vi "Laser Power Control.vi"(7 "Calling VI Ref":refnum<vi>) -> ()   [LabVIEW 2016]
uses:
  Laser Power Control Type Defs/Laser Power Ctrl Main Control.ctl
  Laser Power Control Type Defs/Laser Power Ctrl Setup.ctl
  Hardware Configuration/Hardware Configuration Controls/Device Type.ctl
  <vilib>/Utility/miscctls.llb/LVPointTypeDef.ctl
  Laser Power Control Type Defs/Laser Power Ctrl Settings.ctl
  Hardware Configuration/Hardware Configuration Controls/Device Function.ctl
  Laser Power Control Type Defs/Laser Power Ctrl Notifier Type.ctl
  Laser Power Control Type Defs/Laser Power Ctrl Actions.ctl
  Laser Power Control Type Defs/Laser Power Ctrl Base Type.ctl
  Laser Power Control Type Defs/Laser Power Ctrl Type.ctl
  Device Library/Lasers/Laser Controls/Laser Actions.ctl
  Device Library/AOTFs/AOTF Controls/AOTF Actions.ctl
  Device Library/Lasers/External Power Control/External Power Control Type Defs/External Power Actions.ctl
  Device Manager/Common Device Queue/Common Device Controls/Common Device Actions.ctl
  <vilib>/regexp/Match Regular Expression.xnode
panel:
  in  "Manual Laser Ctrl.":bool
  out "Tab Control":enum32{"Power Adjust", "Setup"}(tab)
  in  "Power Ctrl 04":T1={"Wavelength (nm)"=0, "Active"=TRUE, "Power"=0.0, "Power Slider"=0, "Ctrl Status"=""} {"Power Slider" scale=0.0..100.0}
  in  "Power Ctrl 03":T1={"Wavelength (nm)"=0, "Active"=TRUE, "Power"=0.0, "Power Slider"=0, "Ctrl Status"=""} {"Power Slider" scale=0.0..100.0}
  in  "Power Ctrl 02":T1={"Wavelength (nm)"=0, "Active"=TRUE, "Power"=0.0, "Power Slider"=0, "Ctrl Status"=""} {"Power Slider" scale=0.0..100.0}
  in  "Power Ctrl 01":T1={"Wavelength (nm)"=0, "Active"=TRUE, "Power"=0.0, "Power Slider"=0, "Ctrl Status"=""} {"Power Slider" scale=0.0..100.0}
  in  "Power Ctrl 00":T1={"Wavelength (nm)"=0, "Active"=TRUE, "Power"=0.0, "Power Slider"=0, "Ctrl Status"=""} {"Power Slider" scale=0.0..100.0}
  in  "Power Setup 04":T2 {"Power Control Mode" items=["Direct", "AOTF", "External Ctrl"]}
  in  "Power Setup 03":T2 {"Power Control Mode" items=["Direct", "AOTF", "External Ctrl"]}
  in  "Power Setup 02":T2 {"Power Control Mode" items=["Direct", "AOTF", "External Ctrl"]}
  in  "Power Setup 01":T2 {"Power Control Mode" items=["Direct", "AOTF", "External Ctrl"]}
  in  "Power Setup 00":T2 {"Power Control Mode" items=["Direct", "AOTF", "External Ctrl"]}
  in  "Power Ctrl Setup":bool=TRUE
  in  "Quit":bool
  # "Ctrl Status:"
  # "Ctrl Status:"
  # "Ctrl Status:"
  # "Ctrl Status:"
  # "Ctrl Status:"
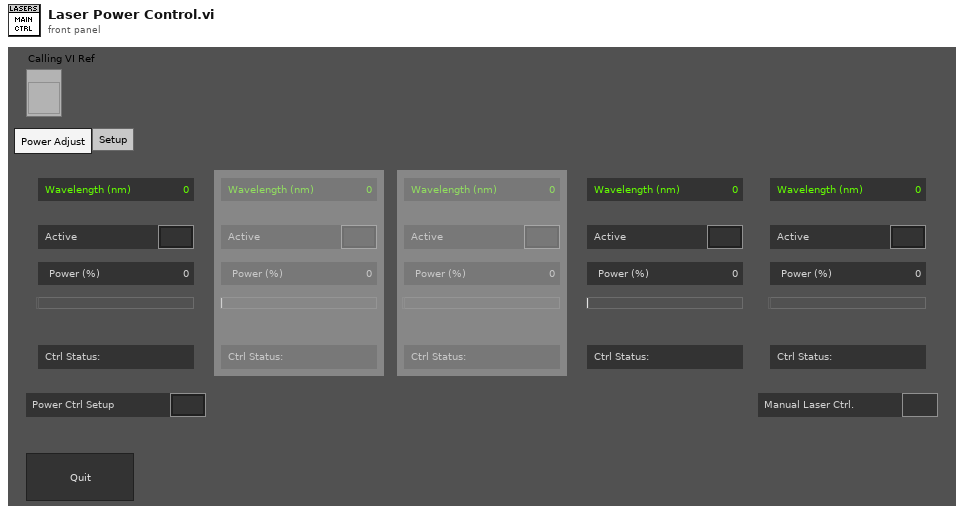
[diagram p1: front panel]
types:
  T1 = typedef "Laser Power Ctrl Main Control.ctl" = cluster{"Wavelength (nm)":u16, "Active":bool, "Power":dbl, "Power Slider":u8, "Ctrl Status":string}
  T2 = typedef "Laser Power Ctrl Setup.ctl" = cluster{"Wavelength (nm)":u16, "Power Control Mode":u16, "Ext Settings":bool, "Ext. Ctrl":string, "Pop Out":bool}
  T3 = typedef "Device Function.ctl" = enum16{"Primary", "Secondary", "Overview", "Wide Field Drift Correction", "642 nm Excitation", "560 nm Excitation", "940 nm Excitation", "546 nm Excitation", "488 nm Excitation", "405 nm Excitation", "Objective Drift Correction", "4Pi Objective Lock", "Objective XY", "Objective Z", "Sample XY", "Sample Coarse Z", "Sample Z", "4Pi Lower", "4Pi Upper", "Mojo", "Adj Cavity", "Line Scanning", "Alert"}
  T4 = typedef "Device Type.ctl" = enum16{"AOTF", "Camera", "Deformable Mirror", "Laser", "Shutter", "Stage", "Waveform", "FPGA", "Email", "Filter Wheel"}
  T5 = typedef "Laser Power Ctrl Settings.ctl" = cluster{"Wavelength":u16, "Ctrl Mode":u16, "Ext Ctrl Path":string, "Settings":string[]}
  T6 = enum16{"Always On", "Always Off", "Off While Running"}
  T7 = typedef "LVPointTypeDef.ctl" = cluster{"Horizontal":i16, "Vertical":i16}
  T8 = typedef "LVRectTypeDef.ctl" = cluster{"Left":i16, "Top":i16, "Right":i16, "Bottom":i16}
  T9 = typedef "LVBoundsTypeDef.ctl" = cluster{"Width":u32, "Height":u32}
  T10 = typedef "Laser Power Ctrl Base Type.ctl" = cluster{"Active":bool, "Power":dbl, "Ctrl Mode":u16}
  T11 = typedef "Laser Power Ctrl Actions.ctl" = enum16{"Exit Loop", "Active", "Power Adj", "All Active On", "All Active Off", "Quit"}
  T12 = typedef "Laser Power Ctrl Notifier Type.ctl" = cluster{"Actions":T11, "Wavelength":u16, "Wavelengths":u16[], "Power Ctrl":T10[]}
  T13 = typedef "Laser Actions.ctl" = enum16{"Error Check", "Set On/Off", "Set Power", "Set Parameter", "Get Power", "Get Status", "Get Parameter", "Quit"}
  T14 = typedef "AOTF Actions.ctl" = enum16{"Error Check", "Blank", "Line On/Off", "Set Power", "Status", "Quit"}
  T15 = typedef "External Power Actions.ctl" = enum16{"Line On/Off", "Set Power", "Set Ctrl Parameters", "Quit"}
  T16 = enum8{"Enabled", "Disabled", "Disabled and Grayed Out"}
  T17 = typedef "Laser Power Ctrl Type.ctl" = enum16{"Direct", "AOTF", "Ext Control"}
  T18 = typedef "Common Device Actions.ctl" = enum16{"Specific Action", "Open Front Panel", "Close Front Panel", "Quit", "Quit All"}
  T19 = cluster{"Wavelength (nm)":bool, "Active":bool, "Power":bool, "Power Slider":bool, "Ctrl Status":bool}
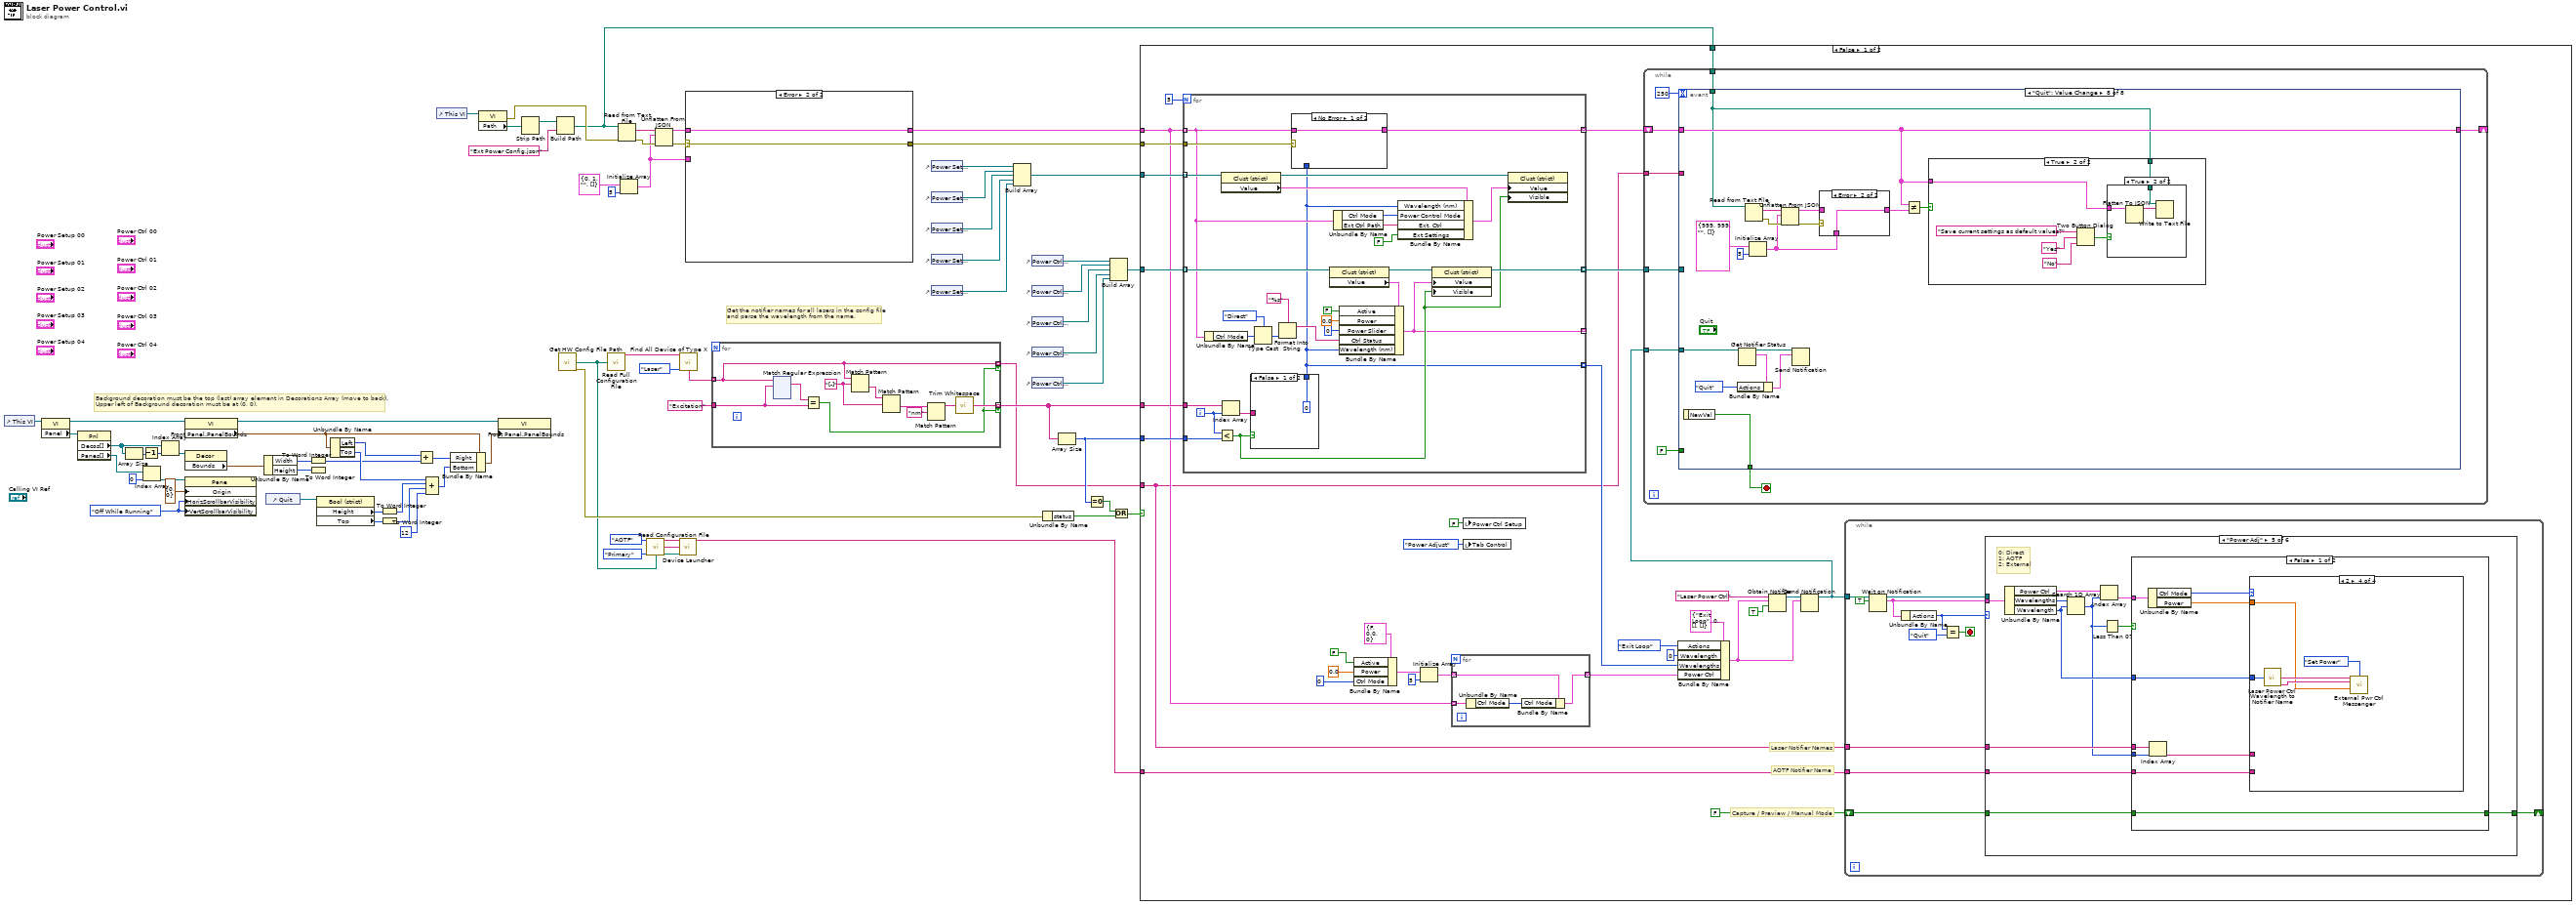
[diagram p0: block diagram]
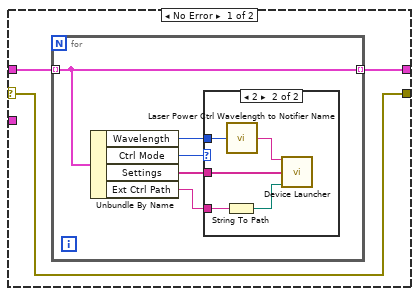
[diagram p2: hidden frame]
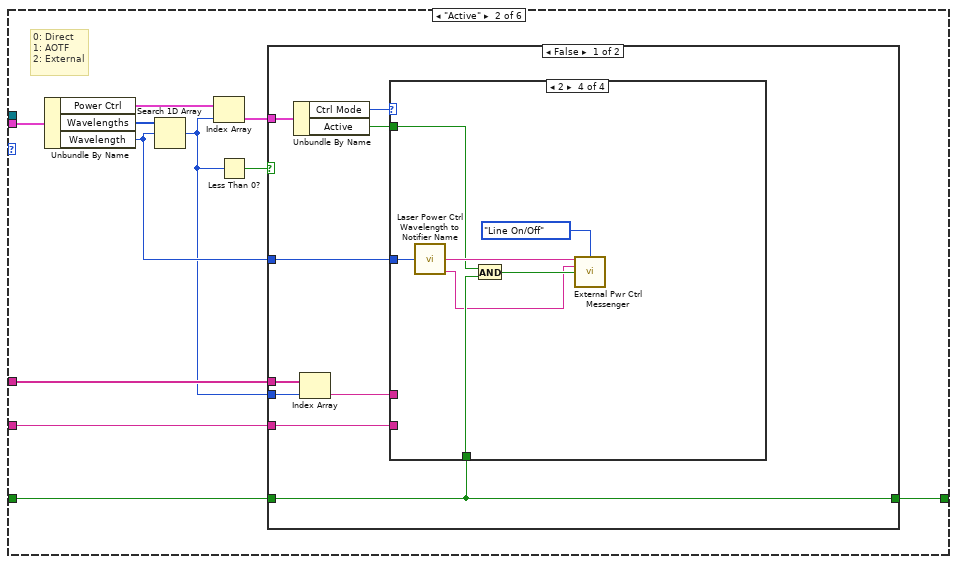
[diagram p5: hidden frame]
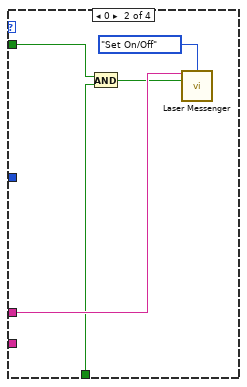
[diagram p7: hidden frame]
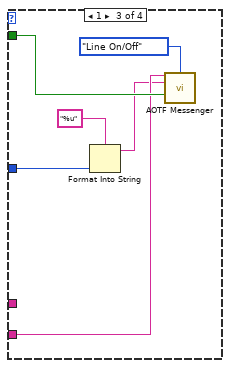
[diagram p8: hidden frame]
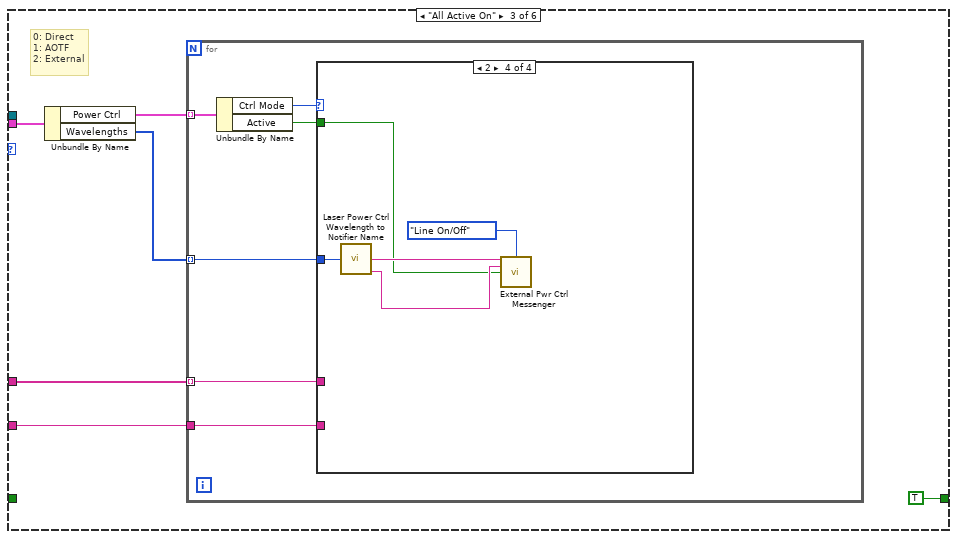
[diagram p10: hidden frame]
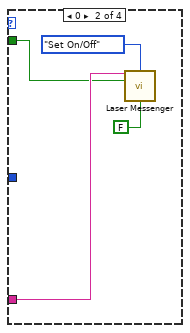
[diagram p12: hidden frame]
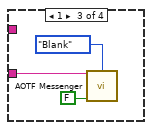
[diagram p13: hidden frame]
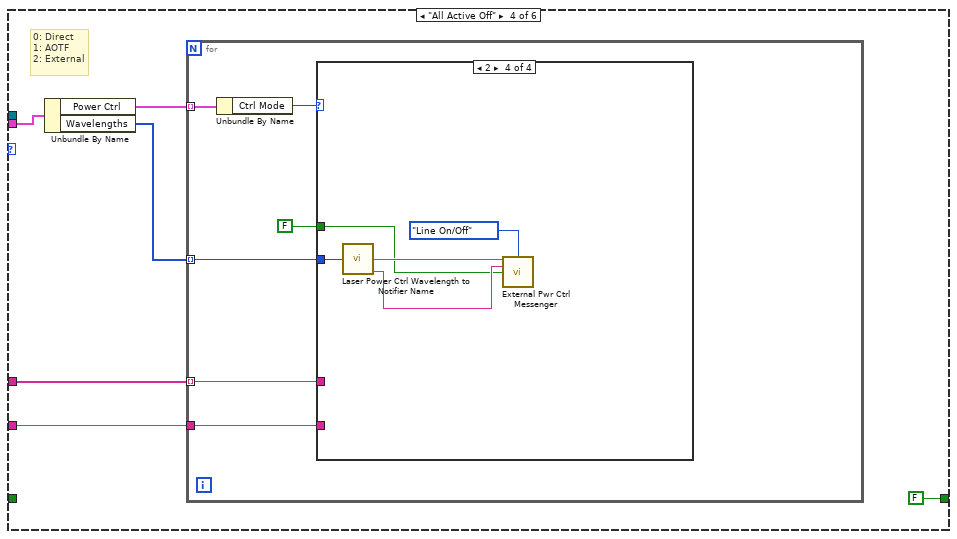
[diagram p14: hidden frame]
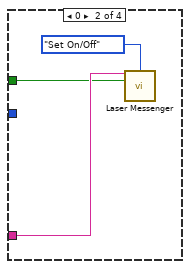
[diagram p16: hidden frame]
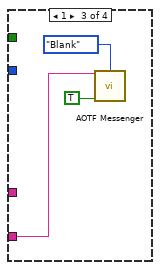
[diagram p17: hidden frame]
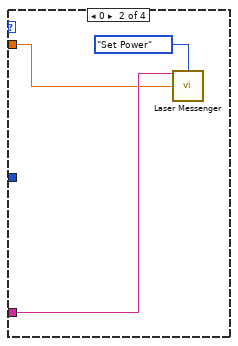
[diagram p19: hidden frame]
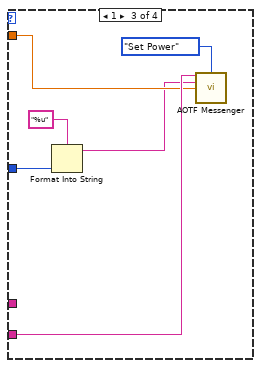
[diagram p20: hidden frame]
diagram:
  w55 = T6."Off While Running" ("Vertical Scrollbar Visibility")
  # "Get the notifier names for all lasers in the config file\nand parse the wavelength from the name."
  # "Background decoration must be the top (last) array element in Decorations Array (move to back).\nUpper left of Background decoration must be at (0, 0)."
  n1 = control-ref of="This VI"() -> (w47:refnum<vi>)
  n2 = property class="VI"(reference=w47) -> (reference out=w56:refnum<vi>, "Panel"=w48:refnum<vi>)  [unwired: 1 in, 1 out]
  n3 = property class="Pnl"(reference=w48) -> ("Decos[]"=w46:refnum<vi>[], "Panes[]"=w52:refnum<vi>[])  [unwired: 1 in, 2 out]
  n4 = Array Size(array=w46) -> (size(s)=w44:i32)
  n5 = Decrement(x=w44) -> (x-1=w45:i32)
  n6 = Index Array(array=w52, index=0) -> (element=w51:refnum<vi>)
  n7 = Index Array(array=w46, index=w45) -> (element=w54:refnum<vi>)
  n8 = property class="VI"(reference=w56) -> (reference out=w58:refnum<vi>, "Front Panel.PanelBounds"=w59:T8)  [unwired: 1 in, 1 out]
  n9 = property class="Decor"(reference=w54) -> ("Bounds"=w57:T9)  [unwired: 1 in, 2 out]
  n10 = property class="Pane"(reference=w51, "Origin"=T7 {"Horizontal"=0, "Vertical"=0}, "HorizScrollbarVisibility"=w55, "VertScrollbarVisibility"=w55) -> ()  [unwired: 1 in, 2 out]
  n11 = Unbundle By Name(w57) -> ("Width"=w62:u32, "Height"=w65:u32)
  n12 = control-ref of="Quit"() -> (w49:refnum<vi>)
  n13 = To Word Integer(number=w62) -> (16bit integer=w64:i16)
  n14 = To Word Integer(number=w65) -> ()  [unwired: 1 out]
  n15 = property class="Bool (strict)"(reference=w49) -> ("Height"=w67:u32, "Top"=w68:i32)  [unwired: 1 in, 2 out]
  n16 = Unbundle By Name(w59) -> ("Left"=w61:i16, "Top"=w72:i16)
  n17 = To Word Integer(number=w67) -> (16bit integer=w70:i16)
  n18 = To Word Integer(number=w68) -> (16bit integer=w71:i16)
  n19 = Add(x=w61, y=w64) -> (x+y=w63:i16)
  n20 = Compound Arithmetic op=ADD(w72, w70, w71, i16 12 ("y")) -> (w66:i16)
  n21 = control-ref of="This VI"() -> (w23:refnum<vi>)
  n22 = Bundle By Name(cluster=w59, "Right"=w63, "Bottom"=w66) -> (w60:T8)
  n23 = property class="VI"(reference=w23) -> (error out=w16:errorcluster, "Path"=w22:path)  [unwired: 1 in, 1 out]
  n24 = property class="VI"(reference=w58, "Front Panel.PanelBounds"=w60) -> ()  [unwired: 1 in, 2 out]
  n25 = Strip Path(path=w22) -> (stripped path=w21:path)  [unwired: 1 out]
  n26 = Build Path(base path=w21, name or relative path="Ext Power Config.json") -> (appended path=w1:path)
  n27 = call "Get HW Config File Path.vi"() -> ("File Path"=w6:path, "Error"=w39:errorcluster)  [unwired: 14 in]
  n28 = call "Read Full Configuration File.vi"("Config File Path"=w6) -> ("Unique Notifier Names"=w74:string[])  [unwired: 11 in, 3 out]
  n29 = Read from Text File(file (use dialog)=w1, error in=w16) -> (text=w19:string, error out=w18:errorcluster)  [unwired: 2 in, 2 out]
  n30 = Initialize Array(T5 {"Wavelength"=0, "Ctrl Mode"=1, "Ext Ctrl Path"="", "Settings"=[]} ("Power Ctrl Settings"), 5 ("dimension size")) -> (w12:T5[])
  n31 = call "Read Configuration File.vi"("Device Type"=Device_Type."AOTF", "Device Function"=Device_Function."Primary", "Config File Path"=w6) -> ("Unique Notifier Name"=w5:string, "Device Ports/IDs/Channels"=w4:string[], "Device Engine Path"=w3:path)  [unwired: 9 in, 1 out]
  n32 = Unflatten From JSON(JSON string=w19, type and defaults=w12, error in (no error)=w18) -> (value=w15:T5[], error out=w17:errorcluster)  [unwired: 4 in]
  n33 = call "Device Launcher.vi"("Notifier Name"=w5, "Device Ports/IDs/Channels"=w4, "Device Engine Path"=w3) -> ("Notifier Name"=w2:string)  [unwired: 11 in, 1 out]
  n34 = call "Find All Device of Type X.vi"("Unique Notifier Names"=w74, "Device Type"=Device_Type."Laser") -> ("All Devices"=w43:string[])  [unwired: 12 in, 1 out]
  n35 = case shown="Error" w17 {
    selector: w17 -> [w75 w88]
    tunnel: w15 -> [w77 _]
    tunnel: [w76 w89] -> w11
    tunnel: w12 -> [_ w89]
    tunnel: [w75 w88] -> w10
    frame No Error {
      n36 = for {
        tunnel: w77 -> [w82] mode=indexing
        tunnel: [w82] -> w76 mode=indexing
        n37 = Unbundle By Name(w82) -> ("Wavelength"=w80:u16, "Ctrl Mode"=w81:u16, "Settings"=w79:string[], "Ext Ctrl Path"=w78:string)
        n38 = case shown="2" w81 {
          tunnel: w80 -> [_ w84]
          tunnel: w79 -> [_ w87]
          tunnel: w78 -> [_ w86]
          frame Default {
          }
          frame 2 {
            n39 = String To Path(string=w86) -> (path=w85:path)
            n40 = call "Laser Power Ctrl Wavelength to Notifier Name.vi"("Wavelength"=w84) -> ("Notifier Name"=w83:string)  [unwired: 13 in, 1 out]
            n41 = call "Device Launcher.vi"("Notifier Name"=w83, "Device Ports/IDs/Channels"=w87, "Device Engine Path"=w85) -> ()  [unwired: 11 in, 2 out]
          }
        }
      }
    }
    frame Error {
    }
  }
  n42 = for {
    tunnel: w43 -> [w97] mode=indexing
    tunnel: [w97] -> w35 mode=indexing if=w90
    tunnel: "Excitation" -> [w98]
    tunnel: [w91] -> w37 mode=indexing if=w90
    w95 = "[-]" ("regular expression")
    n43 = xnode "Match Regular Expression"("input string"=w97, "regular expression"=w98) -> ("whole match"=w99:string)  [unwired: 4 in, 4 out]
    n44 = Equal?(x=w99, y=w98) -> (x = y?=w90:bool)
    n45 = Match Pattern(string=w97, regular expression=w95) -> (after substring=w96:string)  [unwired: 1 in, 3 out]
    n46 = Match Pattern(string=w96, regular expression=w95) -> (after substring=w94:string)  [unwired: 1 in, 3 out]
    n47 = Match Pattern(string=w94, regular expression="nm") -> (before substring=w92:string)  [unwired: 1 in, 3 out]
    n48 = call <vilib>:"Trim Whitespace.vi"("string"=w92) -> ("trimmed string"=w91:string)  [unwired: 1 in]
  }
  n49 = control-ref of="Power Setup 00"() -> (w28:refnum<vi>)
  n50 = control-ref of="Power Setup 01"() -> (w24:refnum<vi>)
  n51 = control-ref of="Power Setup 02"() -> (w25:refnum<vi>)
  n52 = control-ref of="Power Setup 03"() -> (w26:refnum<vi>)
  n53 = control-ref of="Power Setup 04"() -> (w27:refnum<vi>)
  n54 = Build Array(w28, w24, w25, w26, w27) -> (w9:refnum<vi>[])
  n55 = control-ref of="Power Ctrl 00"() -> (w30:refnum<vi>)
  n56 = control-ref of="Power Ctrl 01"() -> (w31:refnum<vi>)
  n57 = control-ref of="Power Ctrl 02"() -> (w32:refnum<vi>)
  n58 = control-ref of="Power Ctrl 03"() -> (w33:refnum<vi>)
  n59 = control-ref of="Power Ctrl 04"() -> (w34:refnum<vi>)
  n60 = Unbundle By Name(w39) -> ("status"=w38:bool)
  n61 = Array Size(array=w37) -> (size(s)=w41:i32)
  n62 = Equal To 0?(x=w41) -> (x = 0?=w40:bool)
  n63 = Build Array(w30, w31, w32, w33, w34) -> (w29:refnum<vi>[])
  n64 = Or(x=w40, y=w38) -> (x .or. y?=w36:bool)
  n65 = case shown="False" w36 {
    tunnel: w41 -> [w245 _]
    tunnel: w37 -> [w244 _]
    tunnel: w35 -> [w218 _]
    tunnel: w29 -> [w242 _]
    tunnel: w9 -> [w241 _]
    tunnel: w11 -> [w225 _]
    tunnel: w10 -> [w240 _]
    tunnel: w2 -> [w219 _]
    tunnel: w1 -> [w214 _]
    frame False {
      # "AOTF Notifier Name"
      # "Laser Notifier Names"
      # "Capture / Preview / Manual Mode"
      n66 = for {
        N: 5 -> [_]
        tunnel: w244 -> [w739]
        tunnel: [w740] -> w243 mode=indexing
        tunnel: w245 -> [w737]
        tunnel: w242 -> [w735] mode=indexing
        tunnel: w241 -> [w729] mode=indexing
        tunnel: w225 -> [w719] mode=indexing
        tunnel: w240 -> [w720]
        tunnel: [w724] -> w221 mode=indexing
        tunnel: [w713] -> _ mode=indexing
        tunnel: [w712] -> w226 mode=indexing
        i -> [w738]
        n67 = Unbundle By Name(w719) -> ("Ctrl Mode"=w714:u16)
        n68 = Less?(x=w738, y=w737) -> (x < y?=w725:bool)
        n69 = property class="Clust (strict)"(reference=w729) -> (reference out=w727:refnum<vi>, "Value"=w728:T2)  [unwired: 1 in, 1 out]
        n70 = Index Array(array=w739, index=w738) -> (element=w736:string)
        n71 = case shown="False" w725 {
          tunnel: [u16 0 ("default value 1") w747] -> w712
          tunnel: w736 -> [_ w746]
          frame False {
          }
          frame True {
            n72 = Scan From String(format string="%u", input string=w746, default 1=u16 0 ("default value 1")) -> (output 1=w747:u16)  [unwired: 2 in, 3 out]
          }
        }
        n73 = Type Cast(type=Laser_Power_Ctrl_Type."Direct" ("Control Mode"), x=w714) -> (*(type *) &x=w716:T17)
        n74 = Format Into String(format string="%s", w716) -> (resulting string=w718:string)  [unwired: 2 in, 1 out]
        n75 = case shown="No Error" w720 {
          tunnel: w719 -> [w741 w744]
          tunnel: w712 -> [_ w743]
          tunnel: [w741 w742] -> w724
          frame No Error {
          }
          frame Error {
            n76 = Bundle By Name(cluster=w744, "Wavelength"=w743) -> (w742:T5)
          }
        }
        n77 = property class="Clust (strict)"(reference=w735) -> (reference out=w734:refnum<vi>, "Value"=w733:T1)  [unwired: 1 in, 1 out]
        n78 = Unbundle By Name(w719) -> ("Ctrl Mode"=w723:u16, "Ext Ctrl Path"=w722:string)
        n79 = Bundle By Name(cluster=w733, "Active"=FALSE, "Power"=0.0 ("Power (%)"), "Power Slider"=u8 0, "Ctrl Status"=w718, "Wavelength (nm)"=w712) -> (w713:T1)
        n80 = Bundle By Name(cluster=w728, "Wavelength (nm)"=w712, "Power Control Mode"=w723, "Ext. Ctrl"=w722, "Ext Settings"=FALSE) -> (w726:T2)
        n81 = property class="Clust (strict)"(reference=w734, "Value"=w713, "Visible"=w725) -> (reference out=w740:refnum<vi>)  [unwired: 1 in, 1 out]
        n82 = property class="Clust (strict)"(reference=w727, "Value"=w726, "Visible"=w725) -> ()  [unwired: 1 in, 2 out]
      }
      n83 = Bundle By Name(cluster=T10 {"Active"=FALSE, "Power"=0.0, "Ctrl Mode"=0} ("Power Ctrl"), "Active"=FALSE, "Power"=0.0, "Ctrl Mode"=u16 0) -> (w229:T10)
      n84 = Initialize Array(w229, 5 ("dimension size")) -> (w224:T10[])
      n85 = for {
        tunnel: w225 -> [w249] mode=indexing
        tunnel: w224 -> [w248] mode=indexing
        tunnel: [w246] -> w223 mode=indexing
        n86 = Unbundle By Name(w249) -> ("Ctrl Mode"=w247:u16)
        n87 = Bundle By Name(cluster=w248, "Ctrl Mode"=w247) -> (w246:T10)
      }
      n88 = local write "Power Ctrl Setup"(FALSE ("Power Ctrl Setup")) -> ()
      n89 = local write "Tab Control"(enum32{"Power Adjust", "Setup"}."Power Adjust" ("Tab Control")) -> ()
      n90 = Bundle By Name(cluster=T12 {"Actions"=enum."Exit Loop", "Wavelength"=0, "Wavelengths"=[], "Power Ctrl"=[]} ("Laser Power Ctrl Note Type"), "Actions"=Laser_Power_Ctrl_Actions."Exit Loop", "Wavelength"=u16 0 ("Index"), "Wavelengths"=w226, "Power Ctrl"=w223) -> (w233:T12)
      n91 = Obtain Notifier(name (unnamed)="Laser Power Ctrl", notification data type=w233, create if not found? (T)=TRUE) -> (notifier out=w239:refnum<notifier>)  [unwired: 1 in, 2 out]
      n92 = Send Notification(notification=w233, notifier=w239) -> (notifier out=w232:refnum<notifier>)  [unwired: 1 in, 1 out]
      n93 = while {
        tunnel: w243 -> [w392]
        tunnel: w232 -> [w389]
        shift-right: [w387] -> _
        shift-left: w221 -> [w388]
        tunnel: w218 -> [w386]
        tunnel: w214 -> [w385]
        stop <- w391 stop-if-true
        n94 = event shown="[7] \"Quit\": Value Change" {
          selector: _ -> [_ _ _ _ _ _ _ _]
          dyn-events: _ -> [_ _ _ _ _ _ _ _]
          timeout: 250 -> [_ _ _ _ _ _ _ _]
          tunnel: w392 -> [w398 w429 _ _ _ _ _ _]
          tunnel: [w400 w454 w564 w601 w619 w677 w683 w700] -> w391
          tunnel: FALSE -> [w400 w454 w564 w601 w619 w677 w683 _]
          tunnel: w389 -> [w397 w421 _ _ w602 w674 _ w699]
          tunnel: w388 -> [w399 w441 w561 w599 w610 w676 w678 w685]
          tunnel: [w399 w438 w557 w599 w610 w676 w678 w685] -> w387
          tunnel: w386 -> [w394 w420 _ _ _ _ _ _]
          tunnel: w385 -> [_ _ _ _ _ _ _ w684]
          event Timeout {
            # "Monitor power for case with direct control (from laser) and for % ctrl (in case outside apps change the power)"
            n95 = event-data() -> ()  [unwired: 1 in, 1 out]
            n96 = Get Notifier Status(notifier=w397) -> (current notification=w396:T12)  [unwired: 1 in, 4 out]
            n97 = Unbundle By Name(w396) -> ("Power Ctrl"=w395:T10[])
            n98 = call "Device Manager Check if Running.vi"() -> ()  [unwired: 15 in, 1 out]
            n99 = for {
              tunnel: w398 -> [w415] mode=indexing
              tunnel: w395 -> [w413] mode=indexing
              tunnel: w394 -> [w406] mode=indexing
              n100 = Unbundle By Name(w413) -> ("Active"=w412:bool, "Power"=w408:dbl, "Ctrl Mode"=w410:u16)
              n101 = property class="Clust (strict)"(reference=w415) -> (reference out=w405:refnum<vi>, "Value"=w414:T1)  [unwired: 1 in, 1 out]
              n102 = case shown="1, 2, Default" w410 {
                tunnel: [0.0 w417] -> w409
                tunnel: w408 -> [_ w417]
                frame 0 {
                }
                frame 1, 2, Default {
                }
              }
              n103 = call "Device Manager Check if Running.vi"("Notifier Name"=w406) -> ("Running?"=w404:bool)  [unwired: 14 in]
              n104 = To Unsigned Byte Integer(number=w409) -> (unsigned 8bit integer=w411:u8)
              n105 = Select(t=T16."Enabled" ("Disabled"), s=w404, f=T16."Disabled and Grayed Out" ("Disabled")) -> (s? t:f=w401:T16)
              n106 = Bundle By Name(cluster=w414, "Active"=w412, "Power"=w409, "Power Slider"=w411) -> (w407:T1)
              n107 = property class="Clust (strict)"(reference=w405, "DisabledEnum"=w401, "Value"=w407) -> ()  [unwired: 1 in, 2 out]
            }
          }
          event Value Change {
            w437 = refnum<vi> refnum  # Generic
            w453 = refnum<vi> refnum  # Generic
            # "This got messy..."
            # "0: Direct\n1: AOTF\n2: External"
            n108 = event-data() -> ("CtlRef"=w442:refnum<vi>, "NewVal"=w444:u16)  [unwired: 1 in]
            n109 = To More Generic Class(target class=w453, reference=w442) -> (generic class reference=w452:refnum<vi>)
            n110 = call "Laser Power Ctrl Index from Name.vi"("Generic Class Ref"=w452) -> ("Index from Name"=w418:i32)  [unwired: 14 in]
            n111 = Index Array(array=w429, index=w418) -> (element=w419:refnum<vi>)
            n112 = Get Notifier Status(notifier=w421) -> (notifier out=w451:refnum<notifier>, current notification=w448:T12)  [unwired: 1 in, 3 out]
            n113 = Index Array(array=w441, index=w418) -> (element=w440:T5)
            n114 = Unbundle By Name(w448) -> ("Power Ctrl"=w446:T10[])
            n115 = case shown="2" w444 {
              selector: w444 -> [w477 w484 _]
              tunnel: w442 -> [w474 w487 w493]
              tunnel: w440 -> [w481 w482 w495]
              tunnel: [w480 w488 w494] -> w439
              tunnel: [w474 w487 w493] -> w435
              tunnel: [FALSE FALSE w492] -> w436
              tunnel: [path "" path "" w491] -> w433
              tunnel: [w477 w484 w490] -> w427
              tunnel: ["Power (mW)" "Power (%)" w489] -> w423
              tunnel: w420 -> [w466 _ _]
              tunnel: w419 -> [w464 _ _]
              tunnel: w418 -> [w460 _ _]
              frame 0, Default {
                w458 = refnum<vi> refnum  # Boolean
                (unwired) refnum<vi> refnum  # Cluster
                w463 = refnum<vi> refnum  # Cluster
                # "Not sure why, but this wont set the value..."
                n116 = Index Array(array=w466, index=w460) -> (element=w465:string)
                n117 = property class="Ring (strict)"(reference=w474) -> ("Owner"=w475:refnum<vi>)  [unwired: 1 in, 2 out]
                n118 = property class="Clust (strict)"(reference=w464) -> ("Controls[]"=w461:refnum<vi>[])  [unwired: 1 in, 2 out]
                n119 = To More Specific Class(target class=w463, reference=w475) -> (specific class reference=w473:refnum<vi>)  [unwired: 1 in, 1 out]
                n120 = property class="Clust"(reference=w473) -> ("Controls[]"=w472:refnum<vi>[])  [unwired: 1 in, 2 out]
                n121 = call "Laser Messenger.vi"("Notifier Name"=w465, "Action"=Laser_Actions."Get Status") -> ("Light Emission?"=w455:bool)  [unwired: 8 in, 5 out]
                n122 = To Variant(anything=w455) -> (Variant=w456:variant)
                n123 = Index Array(array=w472, index=4) -> (element=w470:refnum<vi>)
                n124 = To Variant(anything=TRUE) -> (Variant=w469:variant)
                n125 = property class="Ctl"(reference=w470, "Value"=w469) -> ()  [unwired: 1 in, 2 out]
                n126 = Index Array(array=w461, index=1) -> (element=w459:refnum<vi>)
                n127 = To More Specific Class(target class=w458, reference=w459) -> (specific class reference=w457:refnum<vi>)  [unwired: 1 in, 1 out]
                n128 = property class="Bool"(reference=w457, "Value"=w456) -> ()  [unwired: 1 in, 2 out]
                n129 = Bundle By Name(cluster=w481, "Ctrl Mode"=w477) -> (w480:T5)
              }
              frame 1 {
                # "AOTF"
                n130 = Bundle By Name(cluster=w482, "Ctrl Mode"=w484) -> (w488:T5)
              }
              frame 2 {
                n131 = Unbundle By Name(w495) -> ("Wavelength"=w498:u16, "Ext Ctrl Path"=w505:string, "Settings"=w503:string[])
                n132 = call "Laser Power Ctrl Wavelength to Notifier Name.vi"("Wavelength"=w498) -> ("Notifier Name"=w497:string)  [unwired: 13 in, 1 out]
                n133 = call "Device Manager Check if Running.vi"("Notifier Name"=w497) -> ("Running?"=w507:bool)  [unwired: 14 in]
                n134 = case shown="True" w507 {
                  tunnel: w498 -> [w528 w534]
                  tunnel: [w528 w534] -> w506
                  tunnel: w505 -> [w527 w533]
                  tunnel: [w527 w533] -> w504
                  tunnel: w503 -> [w526 w532]
                  tunnel: [w526 w532] -> w502
                  tunnel: w497 -> [w525 w530]
                  tunnel: [w525 w529] -> w500
                  frame False {
                  }
                  frame True {
                    n135 = call "Common Device Queue Messenger.vi"("Common Action"=Common_Device_Actions."Quit" ("Common Actions"), "Notifier Name"=w530) -> ("Notifier Name"=w529:string)  [unwired: 13 in]
                  }
                }
                n136 = String To Path(string=w504) -> (path=w508:path)
                n137 = call "Laser Power Ctrl Ext Setup.vi"("Wavelength"=w506, "Previous Path"=w508, "Settings"=w502) -> ("Settings Out"=w496:string[], "Ext Ctrl Path"=w501:path, "Canceled?"=w499:bool)  [unwired: 10 in]
                n138 = case shown="False" w499 {
                  tunnel: w501 -> [w511 _]
                  tunnel: w496 -> [w514 _]
                  tunnel: w500 -> [w518 _]
                  tunnel: w493 -> [_ w524]
                  tunnel: [TRUE FALSE] -> w492
                  tunnel: w495 -> [w513 w522]
                  tunnel: [w512 w522] -> w494
                  tunnel: [w511 path ""] -> w491
                  tunnel: [u16 2 ("Ctrl Mode") w520] -> w490
                  tunnel: ["Power (%)" "Power (%)"] -> w489
                  frame False {
                    n139 = Path To String(path=w511) -> (string=w515:string)
                    n140 = call "Device Launcher.vi"("Notifier Name"=w518, "Device Ports/IDs/Channels"=w514, "Device Engine Path"=w511) -> ()  [unwired: 11 in, 2 out]
                    n141 = Bundle By Name(cluster=w513, "Ctrl Mode"=u16 2, "Settings"=w514, "Ext Ctrl Path"=w515) -> (w512:T5)
                  }
                  frame True {
                    w520 = u16 1 ("Value")
                    n142 = property class="Ring (strict)"(reference=w524, "Value"=w520) -> ()  [unwired: 1 in, 2 out]
                  }
                }
              }
            }
            n143 = Index Array(array=w446, index=w418) -> (element=w447:T10)
            n144 = Bundle By Name(cluster=w447, "Ctrl Mode"=w427) -> (w445:T10)
            n145 = Replace Array Subset(array=w446, new element=w445, index=w418) -> (w443:T10[])
            n146 = Bundle By Name(cluster=w448, "Actions"=Laser_Power_Ctrl_Actions."Exit Loop", "Power Ctrl"=w443) -> (w449:T12)
            n147 = Type Cast(type=Laser_Power_Ctrl_Type."Direct" ("Control Mode"), x=w427) -> (*(type *) &x=w431:T17)
            n148 = Send Notification(notification=w449, notifier=w451) -> ()  [unwired: 1 in, 2 out]
            n149 = Format Into String(format string="%s", w431) -> (resulting string=w426:string)  [unwired: 2 in, 1 out]
            n150 = property class="Clust (strict)"(reference=w419) -> (reference out=w425:refnum<vi>, "Value"=w428:T1)  [unwired: 1 in, 1 out]
            n151 = Bundle By Name(cluster=w428, "Ctrl Status"=w426) -> (w424:T1)
            n152 = Replace Array Subset(array=w441, new element=w439, index=w418) -> (w438:T5[])
            n153 = property class="Clust (strict)"(reference=w425, "Value"=w424) -> ("Controls[]"=w422:refnum<vi>[])  [unwired: 1 in, 2 out]
            n154 = To More Generic Class(target class=w437, reference=w435) -> (generic class reference=w434:refnum<vi>)
            n155 = call "Laser Power Ctrl Enable Setup Controls.vi"("Enabled?"=w436, "Generic Class Ref"=w434, "VI Path"=w433) -> ()  [unwired: 13 in]
            n156 = call "Laser Power Ctrl Set Caption.vi"("Caption Text"=w423, "Setup Controls"=w422) -> ()  [unwired: 14 in]
          }
          event Value Change {
            w541 = refnum<vi> refnum  # Cluster
            w563 = refnum<vi> refnum  # Generic
            # "0: Direct\n1: AOTF\n2: External"
            n157 = event-data() -> ("CtlRef"=w538:refnum<vi>)  [unwired: 1 in, 2 out]
            n158 = To More Generic Class(target class=w563, reference=w538) -> (generic class reference=w562:refnum<vi>)
            n159 = property class="Bool (strict)"(reference=w538, "Value"=FALSE) -> ("Owner"=w542:refnum<vi>)  [unwired: 1 in, 2 out]
            n160 = call "Laser Power Ctrl Index from Name.vi"("Generic Class Ref"=w562) -> ("Index from Name"=w559:i32)  [unwired: 14 in]
            n161 = To More Specific Class(target class=w541, reference=w542) -> (specific class reference=w543:refnum<vi>)  [unwired: 1 in, 1 out]
            n162 = Index Array(array=w561, index=w559) -> (element=w560:T5)
            n163 = property class="Clust"(reference=w543) -> ("Controls[]"=w544:refnum<vi>[])  [unwired: 1 in, 2 out]
            n164 = Unbundle By Name(w560) -> ("Wavelength"=w547:u16, "Ext Ctrl Path"=w553:string, "Settings"=w551:string[])
            n165 = for {
              tunnel: w544 -> [w572] mode=indexing
              tunnel: [w569] -> w540
              tunnel: [w568] -> w539
              stop <- w569 stop-if-true
              n166 = property class="Ctl"(reference=w572) -> (reference out=w568:refnum<vi>, "Label.Text"=w571:string)  [unwired: 1 in, 1 out]
              n167 = Equal?(x=w571, y="Ext. Ctrl") -> (x = y?=w569:bool)
            }
            n168 = call "Laser Power Ctrl Wavelength to Notifier Name.vi"("Wavelength"=w547) -> ("Notifier Name"=w546:string)  [unwired: 13 in, 1 out]
            n169 = call "Device Manager Check if Running.vi"("Notifier Name"=w546) -> ("Running?"=w555:bool)  [unwired: 14 in]
            n170 = case shown="True" w555 {
              tunnel: w547 -> [w584 w590]
              tunnel: [w584 w590] -> w554
              tunnel: w553 -> [w583 w589]
              tunnel: [w583 w589] -> w552
              tunnel: w551 -> [w582 w588]
              tunnel: [w582 w588] -> w550
              tunnel: w546 -> [w581 w586]
              tunnel: [w581 w585] -> w549
              frame False {
              }
              frame True {
                n171 = call "Common Device Queue Messenger.vi"("Common Action"=Common_Device_Actions."Quit" ("Common Actions"), "Notifier Name"=w586) -> ("Notifier Name"=w585:string)  [unwired: 13 in]
              }
            }
            n172 = String To Path(string=w552) -> (path=w556:path)
            n173 = call "Laser Power Ctrl Ext Setup.vi"("Wavelength"=w554, "Previous Path"=w556, "Settings"=w550) -> ("Settings Out"=w545:string[], "Ext Ctrl Path"=w537:path, "Canceled?"=w548:bool)  [unwired: 10 in]
            n174 = Strip Path(path=w537) -> (name=w536:string)  [unwired: 1 out]
            n175 = case shown="False" w548 {
              tunnel: w537 -> [w573 _]
              tunnel: w545 -> [w576 _]
              tunnel: w549 -> [w579 _]
              tunnel: w560 -> [w575 w580]
              tunnel: [w574 w580] -> w558
              frame False {
                n176 = Path To String(path=w573) -> (string=w577:string)
                n177 = call "Device Launcher.vi"("Notifier Name"=w579, "Device Ports/IDs/Channels"=w576, "Device Engine Path"=w573) -> ()  [unwired: 11 in, 2 out]
                n178 = Bundle By Name(cluster=w575, "Ctrl Mode"=u16 2, "Settings"=w576, "Ext Ctrl Path"=w577) -> (w574:T5)
              }
              frame True {
              }
            }
            n179 = case shown="False" w540 {
              tunnel: w539 -> [_ w567]
              tunnel: w536 -> [_ w565]
              frame False {
              }
              frame True {
                n180 = To Variant(anything=w565) -> (Variant=w566:variant)
                n181 = property class="Ctl"(reference=w567, "Value"=w566) -> ()  [unwired: 1 in, 2 out]
              }
            }
            n182 = Replace Array Subset(array=w561, new element=w558, index=w559) -> (w557:T5[])
          }
          event Value Change {
            w598 = refnum<vi> refnum  # Generic
            n183 = event-data() -> ("CtlRef"=w600:refnum<vi>)  [unwired: 1 in, 1 out]
            n184 = property class="Bool (strict)"(reference=w600, "Value"=FALSE) -> ()  [unwired: 1 in, 2 out]
            n185 = To More Generic Class(target class=w598, reference=w600) -> (generic class reference=w597:refnum<vi>)
            n186 = call "Laser Power Ctrl Index from Name.vi"("Generic Class Ref"=w597) -> ("Index from Name"=w596:i32)  [unwired: 14 in]
            n187 = Index Array(array=w599, index=w596) -> (element=w594:T5)
            n188 = Unbundle By Name(w594) -> ("Wavelength"=w595:u16)
            n189 = call "Laser Power Ctrl Wavelength to Notifier Name.vi"("Wavelength"=w595) -> ("Notifier Name"=w592:string)  [unwired: 13 in, 1 out]
            n190 = call "Common Device Queue Messenger.vi"("Common Action"=Common_Device_Actions."Open Front Panel" ("Common Actions"), "Notifier Name"=w592) -> ()  [unwired: 13 in, 1 out]
          }
          event Value Change {
            # "Active: 2\nPower (%): 4\nPower Slider: 8"
            n191 = event-data() -> ("NewVal"=w606:T1, "OldVal"=w607:T1, "CtlRef"=w618:refnum<vi>)  [unwired: 1 in]
            n192 = Not Equal?(x=w606, y=w607) -> (x != y?=w609:T19)
            n193 = property class="Clust (strict)"(reference=w618) -> (reference out=w603:refnum<vi>, "Label.Text"=w611:string)  [unwired: 1 in, 1 out]
            n194 = Cluster To Array(cluster=w609) -> (array=w608:bool[])
            n195 = Boolean Array To Number(Boolean array=w608) -> (number=w605:u32)
            n196 = String Length(string=w611) -> (length=w617:i32)
            n197 = Subtract(x=w617, y=2) -> (x-y=w615:i32)
            n198 = String Subset(string=w611, offset (0)=w615) -> (substring=w612:string)  [unwired: 1 in]
            n199 = Scan From String(format string="%u", input string=w612, default 1=0) -> (output 1=w604:i32)  [unwired: 2 in, 3 out]
            n200 = case shown="2" w605 {
              tunnel: w604 -> [_ w624 w638 w656]
              tunnel: w603 -> [_ w633 w650 w667]
              tunnel: w602 -> [_ w623 w636 w654]
              frame Default {
              }
              frame 2 {
                n201 = property class="Clust (strict)"(reference=w633) -> ("Value"=w632:T1)  [unwired: 1 in, 2 out]
                n202 = Unbundle By Name(w632) -> ("Wavelength (nm)"=w621:u16, "Active"=w620:bool)
                n203 = Get Notifier Status(notifier=w623) -> (notifier out=w631:refnum<notifier>, current notification=w629:T12)  [unwired: 1 in, 3 out]
                n204 = Unbundle By Name(w629) -> ("Power Ctrl"=w627:T10[])
                n205 = Index Array(array=w627, index=w624) -> (element=w628:T10)
                n206 = Bundle By Name(cluster=w628, "Active"=w620) -> (w626:T10)
                n207 = Replace Array Subset(array=w627, new element=w626, index=w624) -> (w625:T10[])
                n208 = Bundle By Name(cluster=w629, "Wavelength"=w621, "Power Ctrl"=w625, "Actions"=Laser_Power_Ctrl_Actions."Active") -> (w630:T12)
                n209 = Send Notification(notification=w630, notifier=w631) -> ()  [unwired: 1 in, 2 out]
              }
              frame 4 {
                n210 = property class="Clust (strict)"(reference=w650) -> (reference out=w649:refnum<vi>, "Value"=w648:T1)  [unwired: 1 in, 1 out]
                n211 = Unbundle By Name(w648) -> ("Power"=w637:dbl, "Wavelength (nm)"=w634:u16)
                n212 = To Unsigned Byte Integer(number=w637) -> (unsigned 8bit integer=w647:u8)
                n213 = Get Notifier Status(notifier=w636) -> (notifier out=w645:refnum<notifier>, current notification=w643:T12)  [unwired: 1 in, 3 out]
                n214 = Bundle By Name(cluster=w648, "Power Slider"=w647) -> (w646:T1)
                n215 = Unbundle By Name(w643) -> ("Power Ctrl"=w641:T10[])
                n216 = property class="Clust (strict)"(reference=w649, "Value"=w646) -> ()  [unwired: 1 in, 2 out]
                n217 = Index Array(array=w641, index=w638) -> (element=w642:T10)
                n218 = Bundle By Name(cluster=w642, "Power"=w637) -> (w640:T10)
                n219 = Replace Array Subset(array=w641, new element=w640, index=w638) -> (w639:T10[])
                n220 = Bundle By Name(cluster=w643, "Wavelength"=w634, "Power Ctrl"=w639, "Actions"=Laser_Power_Ctrl_Actions."Power Adj") -> (w644:T12)
                n221 = Send Notification(notification=w644, notifier=w645) -> ()  [unwired: 1 in, 2 out]
              }
              frame 8 {
                n222 = property class="Clust (strict)"(reference=w667) -> (reference out=w666:refnum<vi>, "Value"=w665:T1)  [unwired: 1 in, 1 out]
                n223 = Unbundle By Name(w665) -> ("Power Slider"=w655:u8, "Wavelength (nm)"=w652:u16)
                n224 = To Double Precision Float(number=w655) -> (double precision float=w651:dbl)
                n225 = Get Notifier Status(notifier=w654) -> (notifier out=w663:refnum<notifier>, current notification=w661:T12)  [unwired: 1 in, 3 out]
                n226 = Bundle By Name(cluster=w665, "Power"=w651) -> (w664:T1)
                n227 = Unbundle By Name(w661) -> ("Power Ctrl"=w659:T10[])
                n228 = property class="Clust (strict)"(reference=w666, "Value"=w664) -> ()  [unwired: 1 in, 2 out]
                n229 = Index Array(array=w659, index=w656) -> (element=w660:T10)
                n230 = Bundle By Name(cluster=w660, "Power"=w651) -> (w658:T10)
                n231 = Replace Array Subset(array=w659, new element=w658, index=w656) -> (w657:T10[])
                n232 = Bundle By Name(cluster=w661, "Wavelength"=w652, "Power Ctrl"=w657, "Actions"=Laser_Power_Ctrl_Actions."Power Adj") -> (w662:T12)
                n233 = Send Notification(notification=w662, notifier=w663) -> ()  [unwired: 1 in, 2 out]
              }
            }
          }
          event "Manual Laser Ctrl.": Value Change {
            n234 = event-data() -> ("NewVal"=w671:bool)  [unwired: 1 in]
            n235 = Select(t=Laser_Power_Ctrl_Actions."All Active On" ("Actions"), s=w671, f=Laser_Power_Ctrl_Actions."All Active Off") -> (s? t:f=w669:T11)
            n236 = Get Notifier Status(notifier=w674) -> (notifier out=w675:refnum<notifier>, current notification=w673:T12)  [unwired: 1 in, 3 out]
            n237 = Bundle By Name(cluster=w673, "Actions"=w669) -> (w668:T12)
            n238 = Send Notification(notification=w668, notifier=w675) -> ()  [unwired: 1 in, 2 out]
          }
          event "Power Ctrl Setup": Value Change {
            n239 = event-data() -> ("NewVal"=w682:bool)  [unwired: 1 in]
            n240 = Select(t=enum32{"Power Adjust", "Setup"}."Setup" ("Tab Control"), s=w682, f=enum32{"Power Adjust", "Setup"}."Power Adjust" ("Tab Control")) -> (s? t:f=→"Tab Control":enum32{"Power Adjust", "Setup"})
          }
          event "Quit": Value Change {
            n241 = event-data() -> ("NewVal"=w700:bool)  [unwired: 1 in]
            n242 = Get Notifier Status(notifier=w699) -> (notifier out=w697:refnum<notifier>, current notification=w698:T12)  [unwired: 1 in, 3 out]
            n243 = Bundle By Name(cluster=w698, "Actions"=Laser_Power_Ctrl_Actions."Quit") -> (w695:T12)
            n244 = Read from Text File(file (use dialog)=w684) -> (text=w694:string, error out=w693:errorcluster)  [unwired: 3 in, 2 out]
            n245 = Initialize Array(T5 {"Wavelength"=999, "Ctrl Mode"=999, "Ext Ctrl Path"="", "Settings"=[]} ("Power Ctrl Settings"), 5 ("dimension size")) -> (w688:T5[])
            n246 = Unflatten From JSON(JSON string=w694, type and defaults=w688, error in (no error)=w693) -> (value=w689:T5[], error out=w690:errorcluster)  [unwired: 4 in]
            n247 = Send Notification(notification=w695, notifier=w697) -> ()  [unwired: 1 in, 2 out]
            n248 = case shown="Error" w690 {
              tunnel: w689 -> [w710 _]
              tunnel: [w710 w711] -> w687
              tunnel: w688 -> [_ w711]
              frame No Error {
              }
              frame Error {
              }
            }
            n249 = Not Equal?(x=w685, y=w687) -> (x != y?=w686:bool)
            n250 = case shown="True" w686 {
              tunnel: w685 -> [_ w701]
              tunnel: w684 -> [_ w702]
              frame False {
              }
              frame True {
                n251 = Two Button Dialog(message="Save current settings as default values?", 1:"No" ("F button name (\"Cancel\")"), 2:"Yes" ("T button name (\"OK\")")) -> (T button?=w703:bool)
                n252 = case shown="True" w703 {
                  tunnel: w701 -> [_ w708]
                  tunnel: w702 -> [_ w707]
                  frame False {
                  }
                  frame True {
                    n253 = Flatten To JSON(anything=w708) -> (JSON string=w709:string)  [unwired: 2 in, 1 out]
                    n254 = Write to Text File(file (use dialog)=w707, text=w709) -> ()  [unwired: 2 in, 3 out]
                  }
                }
              }
            }
          }
        }
      }
      n255 = while {
        tunnel: w232 -> [w260]
        shift-right: [w252] -> _
        shift-left: FALSE -> [w253]
        tunnel: w218 -> [w251]
        tunnel: w219 -> [w250]
        stop <- w257 stop-if-true
        n256 = Wait on Notification(notifier=w260, ignore previous (F)=TRUE) -> (notifier out=w254:refnum<notifier>, notification=w255:T12)  [unwired: 2 in, 2 out]
        n257 = Unbundle By Name(w255) -> ("Actions"=w256:T11)
        n258 = Equal?(x=w256, y=Laser_Power_Ctrl_Actions."Quit") -> (x = y?=w257:bool)
        n259 = case shown="\"Power Adj\"" w256 {
          tunnel: w255 -> [_ w271 w306 w330 w357 _]
          tunnel: w254 -> [_ _ _ _ _ w384]
          tunnel: w253 -> [w261 w266 _ _ w352 w383]
          tunnel: [w261 w268 TRUE FALSE w354 w383] -> w252
          tunnel: w251 -> [_ w264 w303 w327 w350 _]
          tunnel: w250 -> [_ w262 w305 w329 w348 _]
          frame "Exit Loop", Default {
          }
          frame "Active" {
            # "0: Direct\n1: AOTF\n2: External"
            n260 = Unbundle By Name(w271) -> ("Power Ctrl"=w270:T10[], "Wavelengths"=w272:u16[], "Wavelength"=w265:u16)
            n261 = Search 1D Array(1D array=w272, element=w265) -> (index of element=w263:i32)  [unwired: 1 in]
            n262 = Index Array(array=w270, index=w263) -> (element=w267:T10)
            n263 = Less Than 0?(x=w263) -> (x < 0?=w269:bool)
            n264 = case shown="False" w269 {
              tunnel: w266 -> [w273 w300]
              tunnel: [w273 w300] -> w268
              tunnel: w267 -> [w281 _]
              tunnel: w265 -> [w275 _]
              tunnel: w264 -> [w279 _]
              tunnel: w263 -> [w278 _]
              tunnel: w262 -> [w276 _]
              frame False {
                n265 = Unbundle By Name(w281) -> ("Ctrl Mode"=w280:u16, "Active"=w274:bool)
                n266 = Index Array(array=w279, index=w278) -> (element=w277:string)
                n267 = case shown="2" w280 {
                  tunnel: w274 -> [_ w283 w291 w296]
                  tunnel: w277 -> [_ w285 _ _]
                  tunnel: w276 -> [_ _ w290 _]
                  tunnel: w275 -> [_ _ w289 w294]
                  tunnel: w273 -> [_ w284 _ w297]
                  frame Default {
                  }
                  frame 0 {
                    n268 = And(x=w283, y=w284) -> (x .and. y?=w282:bool)
                    n269 = call "Laser Messenger.vi"("Notifier Name"=w285, "Action"=Laser_Actions."Set On/Off", "Emission On/Off"=w282) -> ()  [unwired: 7 in, 6 out]
                  }
                  frame 1 {
                    n270 = Format Into String(format string="%u", w289) -> (resulting string=w288:string)  [unwired: 2 in, 1 out]
                    n271 = call "AOTF Messenger.vi"("AOTF Notifier Name"=w290, "AOTF Action"=AOTF_Actions."Line On/Off", "Wavelength (nm)"=w288, "Line On/Off"=w291) -> ()  [unwired: 6 in, 6 out]
                  }
                  frame 2 {
                    n272 = call "Laser Power Ctrl Wavelength to Notifier Name.vi"("Wavelength"=w294) -> ("Notifier Name"=w299:string, "Wavelength"=w293:string)  [unwired: 13 in]
                    n273 = And(x=w296, y=w297) -> (x .and. y?=w298:bool)
                    n274 = call "External Pwr Ctrl Messenger.vi"("Notifier Name"=w299, "Actions"=External_Power_Actions."Line On/Off", "Wavelength"=w293, "Line On/Off"=w298) -> ()  [unwired: 12 in]
                  }
                }
              }
              frame True {
              }
            }
          }
          frame "All Active On" {
            # "0: Direct\n1: AOTF\n2: External"
            n275 = Unbundle By Name(w306) -> ("Power Ctrl"=w302:T10[], "Wavelengths"=w301:u16[])
            n276 = for {
              tunnel: w305 -> [w312]
              tunnel: w303 -> [w309] mode=indexing
              tunnel: w302 -> [w308] mode=indexing
              tunnel: w301 -> [w307] mode=indexing
              n277 = Unbundle By Name(w308) -> ("Ctrl Mode"=w311:u16, "Active"=w310:bool)
              n278 = case shown="2" w311 {
                tunnel: w310 -> [_ w314 _ w320]
                tunnel: w309 -> [_ w315 _ _]
                tunnel: w312 -> [_ _ w318 _]
                tunnel: w307 -> [_ _ _ w321]
                frame Default {
                }
                frame 0 {
                  n279 = call "Laser Messenger.vi"("Notifier Name"=w315, "Action"=Laser_Actions."Set On/Off", "Emission On/Off"=w314, "Exit While Busy (F)?"=FALSE) -> ()  [unwired: 6 in, 6 out]
                }
                frame 1 {
                  n280 = call "AOTF Messenger.vi"("AOTF Notifier Name"=w318, "AOTF Action"=AOTF_Actions."Blank", "Beam Blank"=FALSE) -> ()  [unwired: 7 in, 6 out]
                }
                frame 2 {
                  n281 = call "Laser Power Ctrl Wavelength to Notifier Name.vi"("Wavelength"=w321) -> ("Notifier Name"=w324:string, "Wavelength"=w322:string)  [unwired: 13 in]
                  n282 = call "External Pwr Ctrl Messenger.vi"("Notifier Name"=w324, "Actions"=External_Power_Actions."Line On/Off", "Wavelength"=w322, "Line On/Off"=w320) -> ()  [unwired: 12 in]
                }
              }
            }
          }
          frame "All Active Off" {
            # "0: Direct\n1: AOTF\n2: External"
            n283 = Unbundle By Name(w330) -> ("Power Ctrl"=w326:T10[], "Wavelengths"=w325:u16[])
            n284 = for {
              tunnel: w329 -> [w336]
              tunnel: w327 -> [w334] mode=indexing
              tunnel: w326 -> [w333] mode=indexing
              tunnel: w325 -> [w332] mode=indexing
              n285 = Unbundle By Name(w333) -> ("Ctrl Mode"=w335:u16)
              n286 = case shown="2" w335 {
                tunnel: FALSE -> [_ w337 _ w343]
                tunnel: w334 -> [_ w338 _ _]
                tunnel: w336 -> [_ _ w341 _]
                tunnel: w332 -> [_ _ _ w344]
                frame Default {
                }
                frame 0 {
                  n287 = call "Laser Messenger.vi"("Notifier Name"=w338, "Action"=Laser_Actions."Set On/Off", "Emission On/Off"=w337) -> ()  [unwired: 7 in, 6 out]
                }
                frame 1 {
                  n288 = call "AOTF Messenger.vi"("AOTF Notifier Name"=w341, "AOTF Action"=AOTF_Actions."Blank", "Beam Blank"=TRUE ("Beam Blank 2")) -> ()  [unwired: 7 in, 6 out]
                }
                frame 2 {
                  n289 = call "Laser Power Ctrl Wavelength to Notifier Name.vi"("Wavelength"=w344) -> ("Notifier Name"=w347:string, "Wavelength"=w345:string)  [unwired: 13 in]
                  n290 = call "External Pwr Ctrl Messenger.vi"("Notifier Name"=w347, "Actions"=External_Power_Actions."Line On/Off", "Wavelength"=w345, "Line On/Off"=w343) -> ()  [unwired: 12 in]
                }
              }
            }
          }
          frame "Power Adj" {
            # "0: Direct\n1: AOTF\n2: External"
            n291 = Unbundle By Name(w357) -> ("Power Ctrl"=w356:T10[], "Wavelengths"=w358:u16[], "Wavelength"=w351:u16)
            n292 = Search 1D Array(1D array=w358, element=w351) -> (index of element=w349:i32)  [unwired: 1 in]
            n293 = Index Array(array=w356, index=w349) -> (element=w353:T10)
            n294 = Less Than 0?(x=w349) -> (x < 0?=w355:bool)
            n295 = case shown="False" w355 {
              tunnel: w352 -> [w365 w382]
              tunnel: [w365 w382] -> w354
              tunnel: w353 -> [w367 _]
              tunnel: w351 -> [w360 _]
              tunnel: w350 -> [w364 _]
              tunnel: w349 -> [w363 _]
              tunnel: w348 -> [w361 _]
              frame False {
                n296 = Unbundle By Name(w367) -> ("Ctrl Mode"=w366:u16, "Power"=w359:dbl)
                n297 = Index Array(array=w364, index=w363) -> (element=w362:string)
                n298 = case shown="2" w366 {
                  tunnel: w362 -> [_ w369 _ _]
                  tunnel: w361 -> [_ _ w375 _]
                  tunnel: w360 -> [_ _ w372 w378]
                  tunnel: w359 -> [_ w368 w374 w377]
                  frame Default {
                  }
                  frame 0 {
                    n299 = call "Laser Messenger.vi"("Notifier Name"=w369, "Action"=Laser_Actions."Set Power", "Power (mW)"=w368) -> ()  [unwired: 7 in, 6 out]
                  }
                  frame 1 {
                    n300 = Format Into String(format string="%u", w372) -> (resulting string=w371:string)  [unwired: 2 in, 1 out]
                    n301 = call "AOTF Messenger.vi"("AOTF Notifier Name"=w375, "AOTF Action"=AOTF_Actions."Set Power", "Wavelength (nm)"=w371, "Power (%)"=w374) -> ()  [unwired: 6 in, 6 out]
                  }
                  frame 2 {
                    n302 = call "Laser Power Ctrl Wavelength to Notifier Name.vi"("Wavelength"=w378) -> ("Notifier Name"=w381:string, "Wavelength"=w379:string)  [unwired: 13 in]
                    n303 = call "External Pwr Ctrl Messenger.vi"("Notifier Name"=w381, "Actions"=External_Power_Actions."Set Power", "Wavelength"=w379, "Power (%)"=w377) -> ()  [unwired: 12 in]
                  }
                }
              }
              frame True {
              }
            }
          }
          frame "Quit" {
            n304 = Release Notifier(notifier=w384) -> ()  [unwired: 2 in, 3 out]
          }
        }
      }
    }
    frame True {
    }
  }
